vi "Compare Folders.vi"(6 "Folders to Exclude":string[](array[string]), 8 "error in (no error)":errorcluster, 10 "Folder 2":path, 11 "Folder 1":path) -> (0 "error out":errorcluster, 3 "Folder Shot Results":T1)   [LabVIEW 2016, in "SLL File IO.lvlib"]
doc: "Compare two folders and provide the list of \n1. Files Modified\n2. Files Deleted\n3. Files Added\n\nThis uses CRC check to validate if the files have been modiied or not."
uses:
  SLL File IO.lvlib
  _Typedefs/Folder Shot Result.ctl
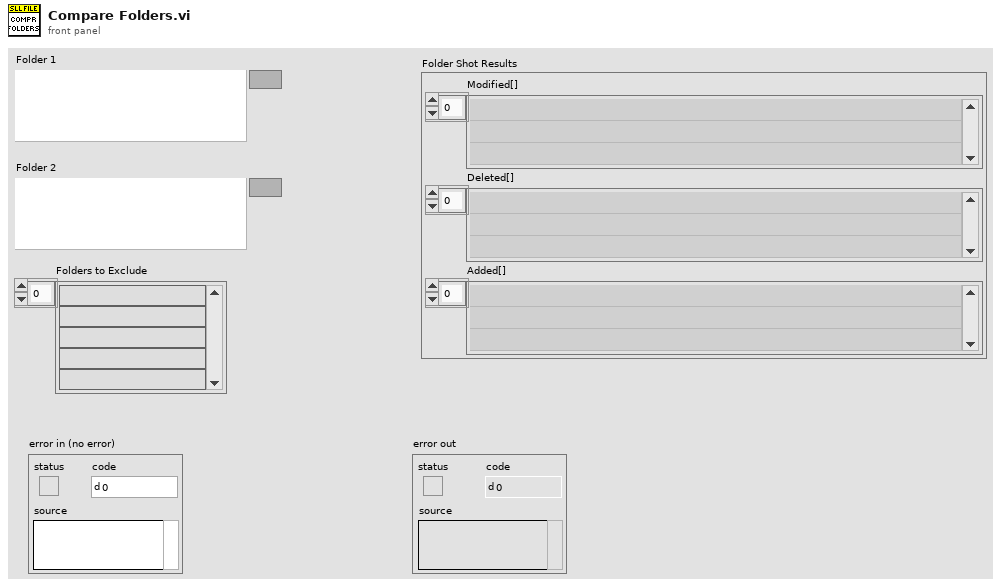
[diagram p1: front panel]
types:
  T1 = typedef "SLL File IO.lvlib/Folder Shot Result.ctl" = cluster{"Modified[]":path[], "Deleted[]":path[], "Added[]":path[]}
  T2 = typedef "SLL File IO.lvlib/Folder Shot Element.ctl" = cluster{"Abs.Path":path, "Relative Path":path, "MD5":string}
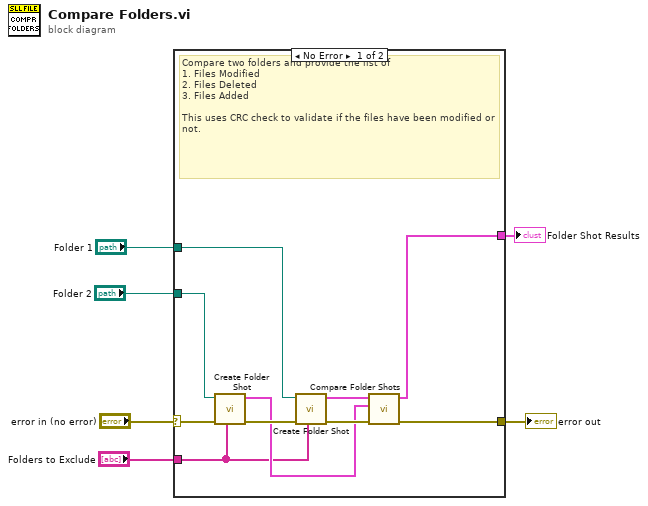
[diagram p0: block diagram]
diagram:
  n1 = case shown="No Error" "error in (no error)" {
    selector: "error in (no error)" -> [w16 w17]
    tunnel: [w11 w17] -> w5
    tunnel: "Folder 2" -> [w14 _]
    tunnel: "Folder 1" -> [w12 _]
    tunnel: [w8 _] -> w1
    tunnel: "Folders to Exclude" -> [w7 _]
    frame No Error {
      # "Compare two folders and provide the list of \n1. Files Modified\n2. Files Deleted\n3. Files Added\n\nThis uses CRC check to validate if the files have been modified or not."
      n2 = call "Create Folder Shot.vi"("Folders to Exclude"=w7, "error in (no error)"=w16, "Directory Path"=w14) -> ("error out"=w15:errorcluster, "Folder Shot"=w9:T2[])  [unwired: 7 in]
      n3 = call "Create Folder Shot.vi"("Folders to Exclude"=w7, "error in (no error)"=w15, "Directory Path"=w12) -> ("error out"=w13:errorcluster, "Folder Shot"=w10:T2[])  [unwired: 7 in]
      n4 = call "Compare Folder Shots.vi"("error in (no error)"=w13, "Folder Shot 2"=w9, "Folder Shot 1"=w10) -> ("error out"=w11:errorcluster, "Folder Shot Results"=w8:T1)  [unwired: 7 in]
    }
    frame Error {
    }
  }
  "error out" <- w5
  "Folder Shot Results" <- w1
